vi "mupExpr Plot.vi"() -> ()   [LabVIEW 2015]
uses:
  <vilib>/Utility/error.llb/DialogType.ctl
  mupExpr/mupExpr.lvclass
  mupExpr/mupExpr.lvclass/mupExpr.ctl
  mupExpr/Eval_SglVar_BulkMode.vi
  mupLib/mupEvalBulk.vi
  mupLib/mupSetVarValue_Array.vi
  mupLib/mupCheckError.vi
  mupLib/mupLibPath.vi
  <vilib>/Utility/error.llb/Error Cluster From Error Code.vi
panel:
  in  "Expression":string="sin(x)"
  in  "Increment":dbl=0.01
  in  "Start":dbl
  in  "End":dbl=6.283
  in  "Plot":bool
  out "XY Graph":cluster{dbl[], "Result":dbl[]}(graph)
  # "Single Variable \"x\""
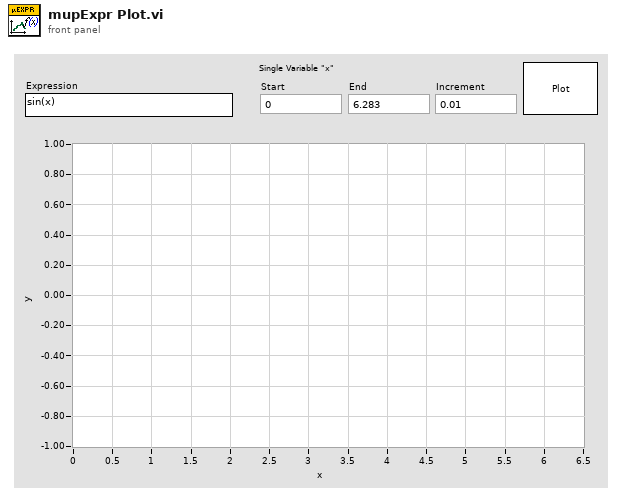
[diagram p1: front panel]
types:
  T1 = typedef "DialogType.ctl" = u16
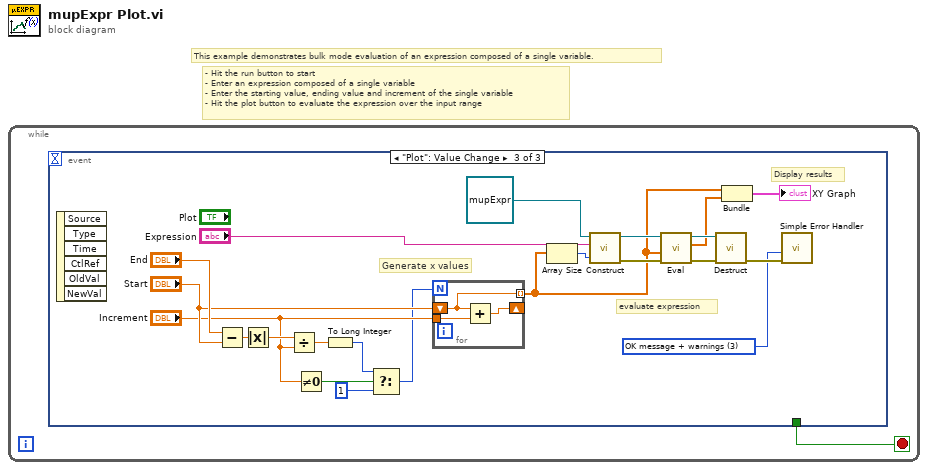
[diagram p0: block diagram]
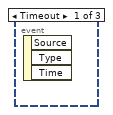
[diagram p2: hidden frame]
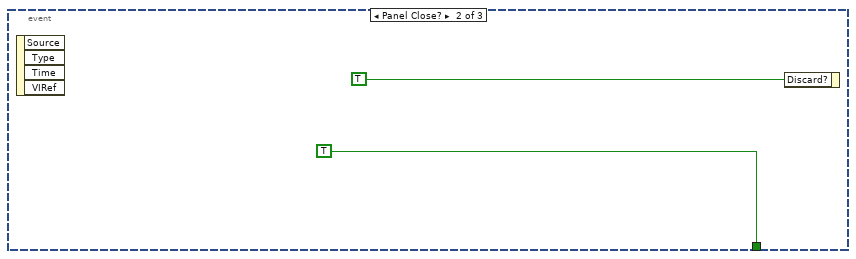
[diagram p3: hidden frame]
diagram:
  # "- Hit the run button to start\n- Enter an expression composed of a single variable\n- Enter the starting value, ending value and increment of the single variable\n- Hit the plot button to evaluate the expression over the input range"
  # "This example demonstrates bulk mode evaluation of an expression composed of a single variable."
  n1 = while {
    stop <- w1 stop-if-true
    n2 = event shown="[2] \"Plot\": Value Change" {
      selector: _ -> [_ _ _]
      dyn-events: _ -> [_ _ _]
      timeout: _ -> [_ _ _]
      tunnel: [_ TRUE _] -> w1
      event Timeout {
        n3 = event-data() -> ()  [unwired: 1 in, 3 out]
      }
      event Panel Close? {
        n4 = event-data() -> ()  [unwired: 1 in, 4 out]
        n5 = event-data("Discard?"=TRUE) -> ()  [unwired: 1 in, 1 out]
      }
      event "Plot": Value Change {
        w10 = T1 3 items=["no dialog", "OK message", "continue or stop message", "OK message + warnings", "continue/stop + warnings"] ("type of dialog (OK msg:1)")
        # "Display results"
        # "evaluate expression"
        # "Generate x values"
        n6 = event-data() -> ()  [unwired: 1 in, 6 out]
        n7 = Subtract(x="End", y="Start") -> (x-y=w22:dbl)
        n8 = Absolute Value(x=w22) -> (abs(x)=w23:dbl)
        n9 = Divide(x=w23, y="Increment") -> (x/y=w24:dbl)
        n10 = Not Equal To 0?(x="Increment") -> (x != 0?=w21:bool)
        n11 = To Long Integer(number=w24) -> (32bit integer=w20:i32)
        n12 = Select(t=w20, s=w21, f=1) -> (s? t:f=w7:i32)
        n13 = for {
          N: w7 -> [_]
          tunnel: "Increment" -> [w28]
          shift-right: [w27] -> _
          shift-left: "Start" -> [w26]
          tunnel: [w26] -> w6 mode=indexing
          n14 = Add(x=w26, y=w28) -> (x+y=w27:dbl)
        }
        n15 = Array Size(array=w6) -> (size(s)=w5:i32)
        n16 = call-dynamic "Construct.vi"("Bulk Size (1)"=w5, "Expression"="Expression", "muExpr in"=refnum<class "mupExpr.lvclass"> refnum) -> ("error out"=w14:errorcluster, "mupExpr out"=w15:refnum<class "mupExpr.lvclass">)  [unwired: 5 in, 2 out]
        n17 = call-poly "Eval.vi"("error in (no error)"=w14, "varValue"=w6, "muExpr in"=w15) -> ("error out"=w12:errorcluster, "Result"=w9:dbl[], "muExpr out"=w13:refnum<class "mupExpr.lvclass">)  [unwired: 6 in]
        n18 = call-dynamic "Destruct.vi"("error in (no error)"=w12, "muExpr in"=w13) -> ("error out"=w11:errorcluster)  [unwired: 9 in]
        n19 = Bundle(w6, "Result"=w9) -> (→"XY Graph":cluster{dbl[], "Result":dbl[]})  [unwired: 1 in]
        n20 = call <vilib>:"Simple Error Handler.vi"("type of dialog (OK msg:1)"=w10, "error in (no error)"=w11) -> ()  [unwired: 3 in, 5 out]
      }
    }
  }
